vi "query TDF File On.vi"(8 "error in (no error)":errorcluster caption="에러 입력(에러 없음)", 10 "File Name":string, 11 "FSV-40N 입력":refnum<class "FSV-40N.lvclass">) -> (0 "error out":errorcluster caption="에러 출력", 2 "On?":bool, 3 "FSV-40N 출력":refnum<class "FSV-40N.lvclass">)   [LabVIEW 2023, in "Spectrum Analyzer.lvlib" / "FSV-40N.lvclass"]
uses:
  FSV-40N.lvclass
  FSV-40N.lvclass/FSV-40N.ctl
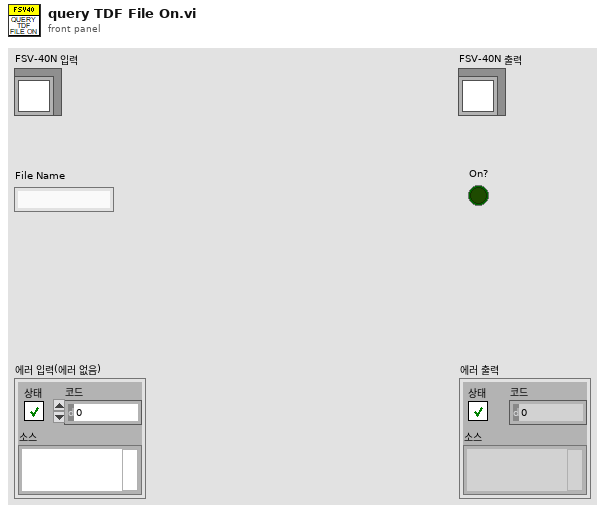
[diagram p1: front panel]
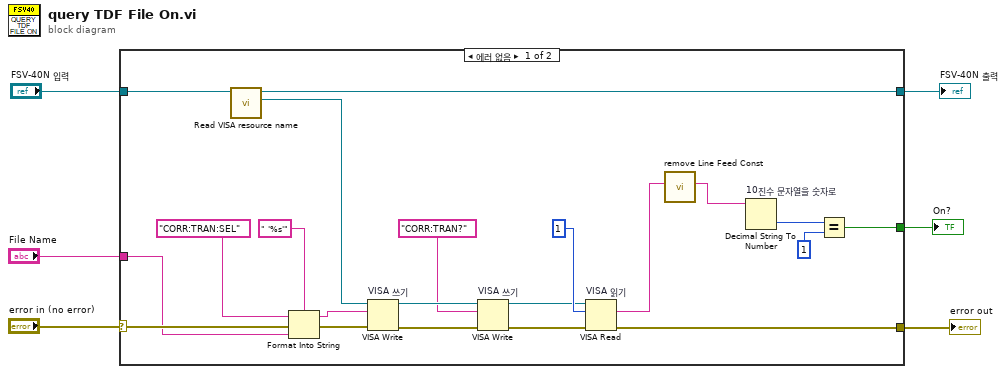
[diagram p0: block diagram]
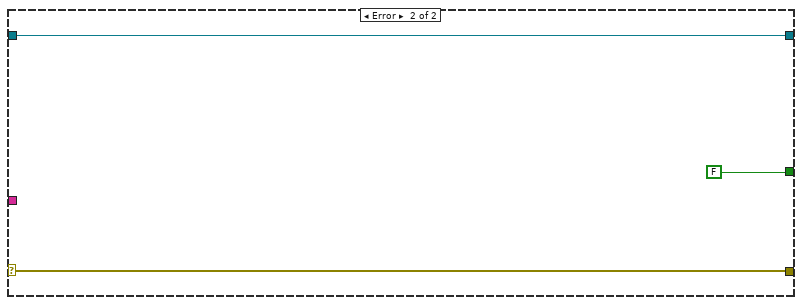
[diagram p2: hidden frame]
diagram:
  n1 = case shown="에러 없음" "error in (no error)" {
    selector: "error in (no error)" -> [w27 w28]
    tunnel: "FSV-40N 입력" -> [w26 w29]
    tunnel: "File Name" -> [w25 _]
    tunnel: [w9 w29] -> w3
    tunnel: [w8 FALSE] -> w2
    tunnel: [w7 w28] -> w1
    frame No Error {
      n2 = call "Read VISA resource name.vi"("FSV-40N in"=w26) -> ("VISA resource name"=w21:refnum<visa-resource-name>, "FSV-40N out"=w9:refnum<class "FSV-40N.lvclass">)  [unwired: 8 in, 1 out]
      n3 = Format Into String(format string=" '%s'" ("포맷 문자열"), initial string="CORR:TRAN:SEL" ("초기 문자열"), error in=w27, w25) -> (resulting string=w20:string, error out=w22:errorcluster)
      n4 = VISA Write "VISA 쓰기"(VISA resource name=w21, write buffer=w20, error in (no error)=w22) -> (VISA resource name out=w18:refnum<visa-resource-name>, error out=w19:errorcluster)  [unwired: 1 out]
      n5 = VISA Write "VISA 쓰기"(VISA resource name=w18, write buffer="CORR:TRAN?" ("버퍼 쓰기"), error in (no error)=w19) -> (VISA resource name out=w14:refnum<visa-resource-name>, error out=w16:errorcluster)  [unwired: 1 out]
      n6 = VISA Read "VISA 읽기"(VISA resource name=w14, byte count=u32 1 ("바이트 카운트"), error in (no error)=w16) -> (read buffer=w13:string, error out=w7:errorcluster)  [unwired: 2 out]
      n7 = call "remove Line Feed Const.vi"("Input"=w13) -> ("Output"=w12:string)  [unwired: 10 in]
      n8 = Decimal String To Number "10진수 문자열을 숫자로"(string=w12) -> (number=w11:i32)  [unwired: 2 in, 1 out]
      n9 = Equal?(x=w11, y=1) -> (x = y?=w8:bool)
    }
    frame Error {
    }
  }
  "error out" <- w1
  "FSV-40N 출력" <- w3
  "On?" <- w2
